vi "Config_Path.vi"(8 "error in (no error)":errorcluster caption="错误输入（无错误）", 11 "Path_management 输入":refnum<class "Path_management.lvclass">) -> (0 "error out":errorcluster caption="错误输出", 2 "添加的路径":path, 3 "Path_management 输出":refnum<class "Path_management.lvclass">)   [LabVIEW 2025, in "Path_management.lvclass"]
uses:
  Path_management.lvclass
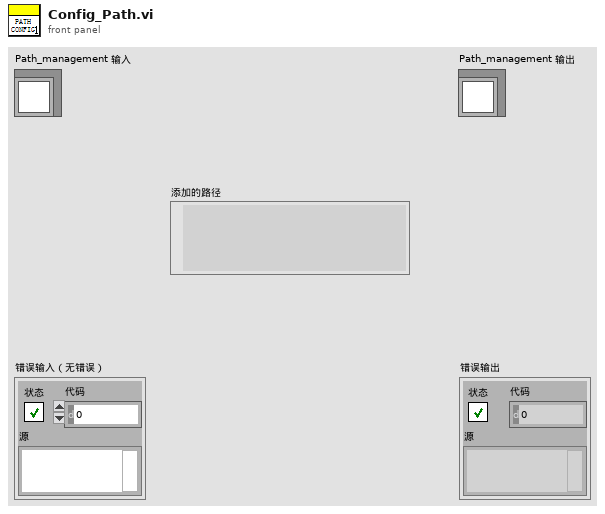
[diagram p1: front panel]
types:
  T1 = enum32{"invalid app kind", "Development System", "Run Time System", "Student Edition", "Embedded LabVIEW", "Evaluation", "Custom"}
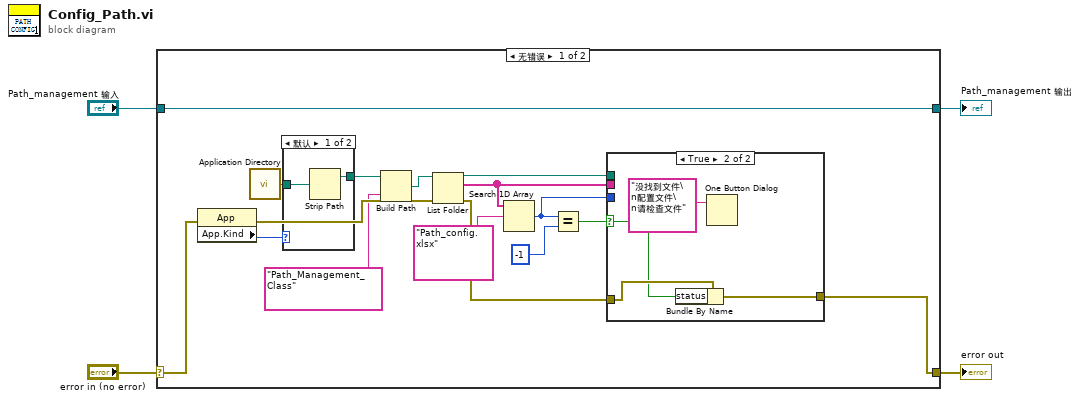
[diagram p0: block diagram]
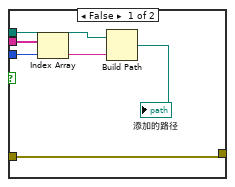
[diagram p3: hidden frame]
diagram:
  n1 = case shown="无错误" "error in (no error)" {
    selector: "error in (no error)" -> [w11 w35]
    tunnel: [w8 w35] -> w3
    tunnel: [w20 w34] -> w1
    tunnel: "Path_management 输入" -> [w20 w34]
    frame No Error {
      n2 = property class="App"(error in=w11) -> (error out=w10:errorcluster, "App.Kind"=w13:T1)  [unwired: 1 in, 1 out]
      n3 = call <vilib>:"Application Directory.vi"() -> ("Application Directory"=w14:path)
      n4 = case shown="默认" w13 {
        tunnel: [w22 w23] -> w7
        tunnel: w14 -> [w21 w23]
        frame Default {
          n5 = Strip Path(path=w21) -> (stripped path=w22:path)  [unwired: 1 out]
        }
        frame "Development System" {
        }
      }
      n6 = Build Path(base path=w7, name or relative path="Path_Management_Class" ("名称或相对路径")) -> (appended path=w6:path)
      n7 = List Folder(path=w6, error in=w10) -> (path out=w17:path, filenames=w19:string[], error out=w9:errorcluster)  [unwired: 2 in, 1 out]
      n8 = Search 1D Array(1D array=w19, element="Path_config.xlsx" ("元素")) -> (index of element=w16:i32)  [unwired: 1 in]
      n9 = Equal?(x=w16, y=-1) -> (x = y?=w12:bool)
      n10 = case shown="True" w12 {
        selector: w12 -> [_ w31]
        tunnel: w19 -> [w29 _]
        tunnel: w17 -> [w27 _]
        tunnel: w16 -> [w26 _]
        tunnel: w9 -> [w25 w32]
        tunnel: [w25 w30] -> w8
        frame False {
          n11 = Index Array(array=w29, index=w26) -> (element=w28:string)
          n12 = Build Path(base path=w27, name or relative path=w28) -> (appended path=→"添加的路径":path)
        }
        frame True {
          n13 = Bundle By Name(cluster=w32, "status"=w31) -> (w30:errorcluster)
          n14 = One Button Dialog(message="没找到文件\n配置文件\n请检查文件" ("消息")) -> ()  [unwired: 1 in, 1 out]
        }
      }
    }
    frame Error {
    }
  }
  "error out" <- w3
  "Path_management 输出" <- w1
